vi "RichToFlatauth_LogoutRequest.vi"(5 "OutputClusterType":T1, 11 "InputCluster":T2) -> (3 "OutputCluster":T1)   [LabVIEW 2020, in "grpc-auth_client.lvlib"]
uses:
  grpc-auth_client.lvlib
  auth_LogoutRequest.ctl
  auth_LogoutRequest_Flat.ctl
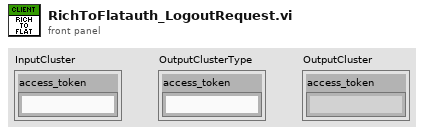
[diagram p1: front panel]
types:
  T1 = typedef "grpc-auth_client.lvlib/auth_LogoutRequest_Flat.ctl" = cluster{"access_token":string}
  T2 = typedef "grpc-auth_client.lvlib/auth_LogoutRequest.ctl" = cluster{"access_token":string}
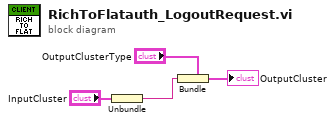
[diagram p0: block diagram]
diagram:
  n1 = Unbundle "Unbundle"("InputCluster") -> ("access_token"=w1:string)
  n2 = Bundle "Bundle"(cluster="OutputClusterType", "access_token"=w1) -> (→"OutputCluster":T1)
